vi "Read Folder Shot File.vi"(8 "error in (no error)":errorcluster, 11 "Log Path":path) -> (0 "error out":errorcluster, 3 "Folder Shot":T1[](array[typedef]))   [LabVIEW 2016, in "SLL File IO.lvlib"]
doc: "Reads a Folder Shot file and returns the Folder Shot Cluster Array."
uses:
  SLL File IO.lvlib
  _Typedefs/Folder Shot Element.ctl
  <vilib>/Utility/file.llb/Read Delimited Spreadsheet (string).vi
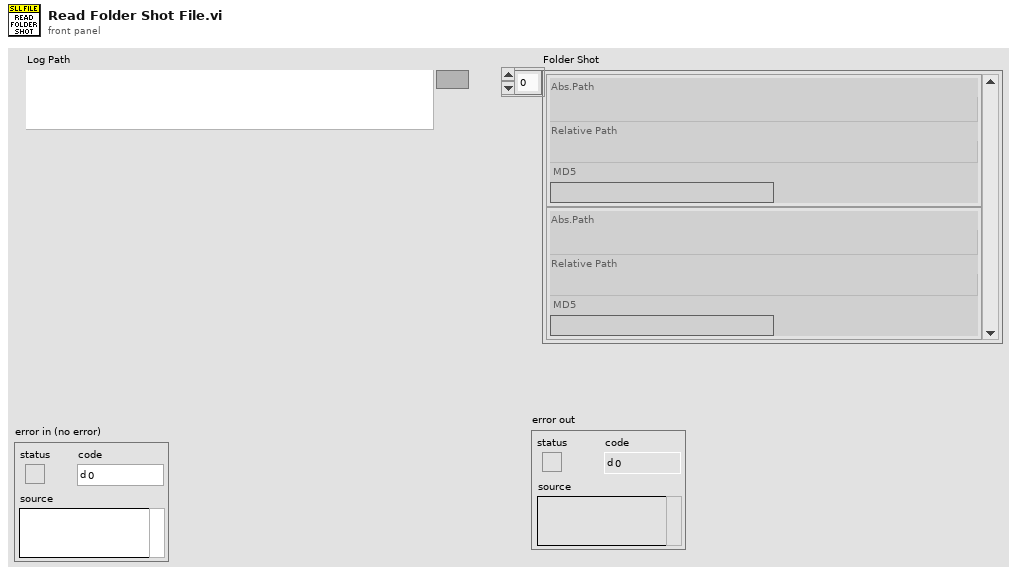
[diagram p1: front panel]
types:
  T1 = typedef "SLL File IO.lvlib/Folder Shot Element.ctl" = cluster{"Abs.Path":path, "Relative Path":path, "MD5":string}
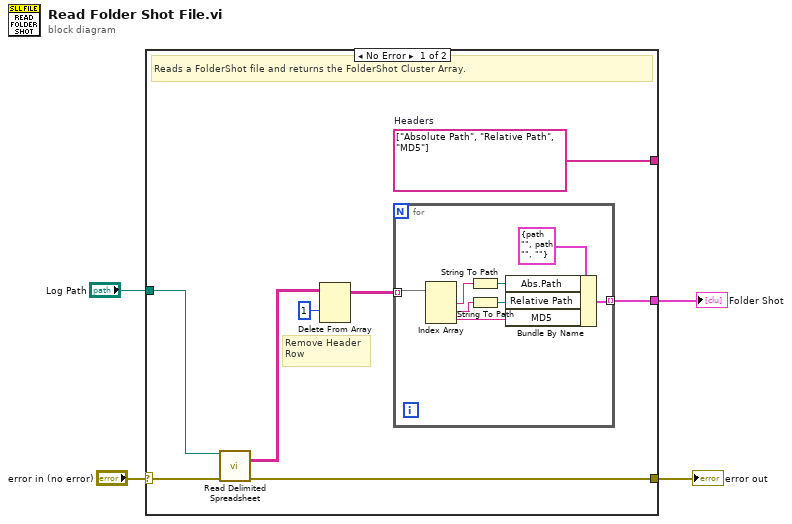
[diagram p0: block diagram]
diagram:
  n1 = case shown="No Error" "error in (no error)" {
    selector: "error in (no error)" -> [w7 w21]
    tunnel: [w8 w21] -> w3
    tunnel: "Log Path" -> [w12 _]
    tunnel: [w9 _] -> w1
    tunnel: [w5 _] -> _
    frame No Error {
      w5 = string[] ["Absolute Path", "Relative Path", "MD5"]  # Headers
      # "Remove Header\nRow"
      # "Reads a FolderShot file and returns the FolderShot Cluster Array."
      n2 = call-poly <vilib>:"Read Delimited Spreadsheet.vi"("file path (dialog if empty)"=w12, "error in (no error)"=w7) -> ("all rows"=w6:string[][], "error out"=w8:errorcluster)  [unwired: 8 in, 4 out]
      n3 = Delete From Array(array=w6, index (row)=1) -> (array with subset deleted=w10:string[][])  [unwired: 2 in, 1 out]
      n4 = for {
        tunnel: w10 -> [w20] mode=indexing
        tunnel: [w13] -> w9 mode=indexing
        n5 = Index Array(array=w20) -> (element #1=w17:string, element #2=w15:string, element #3=w18:string)  [unwired: 3 in]
        n6 = String To Path(string=w17) -> (path=w16:path)
        n7 = String To Path(string=w15) -> (path=w14:path)
        n8 = Bundle By Name(cluster=T1 {"Abs.Path"=path "", "Relative Path"=path "", "MD5"=""} ("Folder Shot Element"), "Abs.Path"=w16, "Relative Path"=w14, "MD5"=w18) -> (w13:T1)
      }
    }
    frame Error {
    }
  }
  "error out" <- w3
  "Folder Shot" <- w1
